vi "[ex ce] Ordinary Differential Equations.vi"(6 "time variable":string="t", 7 "time end":dbl=5.0 format="%.2f", 10 "h (time step)":dbl=0.001 min=0.0 format="%.4f", 11 "time start":dbl format="%.2f") -> (1 "GMath ticks":u32 caption="ms")   [LabVIEW 2021]
doc: "CE-Math example.\n\n::: CalcExpress Toolkit :::\nCopyright (c) 2000-2026 Konstantin Shifershteyn. All rights reserved."
uses:
  ce exmpl - 2D difference info.ctl
  <vilib>/gmath/NI_Gmath.lvlib
panel:
  out "max relative difference":T1 {"relative difference, %" format="%#.6g"; "absolute difference" format="%#.6g"}
  out "max absolute difference":T1 {"relative difference, %" format="%#.6g"; "absolute difference" format="%#.6g"}
  in  "stop":bool
  in  "calc":bool
  in  "example":u16(ring) items=["three equations", "two equations", "one equation"]
  out "speed ratio":dbl format="%.3f"
  out "CE stat":string
  out "GM stat":string
  in  "method":enum16{"Runge Kutta", "Euler"}(ring)
  in  "equation parameters":T2(array[cluster])=[{"variable"="x", "formula"="10*(y-x)", "init value"=1.0}, {"variable"="y", "formula"="x*(28-z)-y", "init value"=1.0}, {"variable"="z", "formula"="x*y-(8/3)*z", "init value"=1.0}] {"init value" format="%.2f"}
  out "CalcExpress ticks":u32 caption="ms"
  out "CE data":cluster{dbl[], dbl[]}[](graph) caption="CalcExpress solution"
  out "GM data":cluster{dbl[], dbl[]}[](graph) caption="G Math solution"
  # "NOTE    CalcExpress uses (^) operator to perform bitwise-XOR operation but not exponentiation operation.\nYou have to use double-asterisk (**) operator to compute an exponent in a CalcExpress expression. For sample, x**y ."
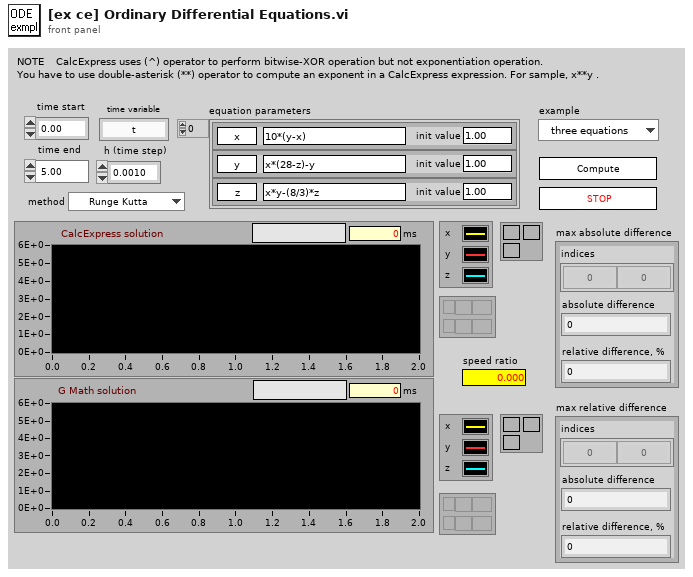
[diagram p1: front panel]
types:
  T1 = typedef "ce exmpl - 2D difference info.ctl" = cluster{"indices":i32[], "absolute difference":dbl, "relative difference, %":dbl}
  T2 = cluster{"variable":string, "formula":string, "init value":dbl}[]
  T3 = cluster{"indexes":i32[], "absolute difference":dbl, "relative difference, %":dbl}
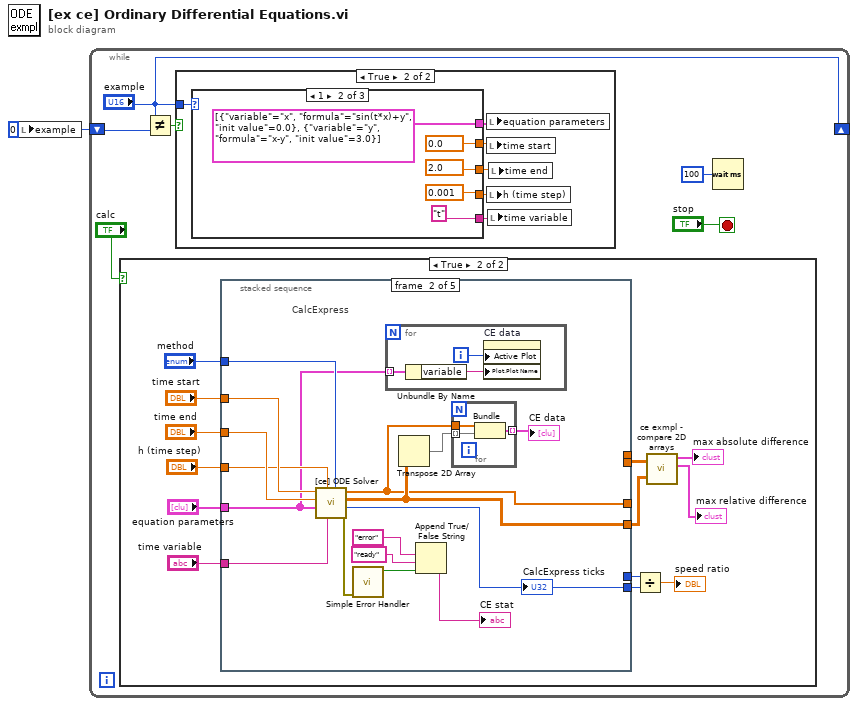
[diagram p0: block diagram]
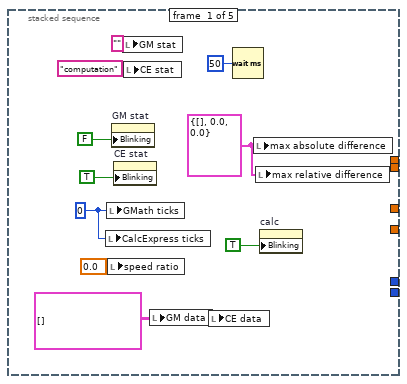
[diagram p3: hidden frame]
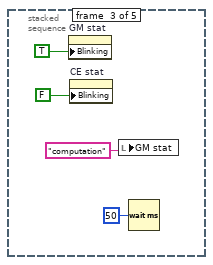
[diagram p4: hidden frame]
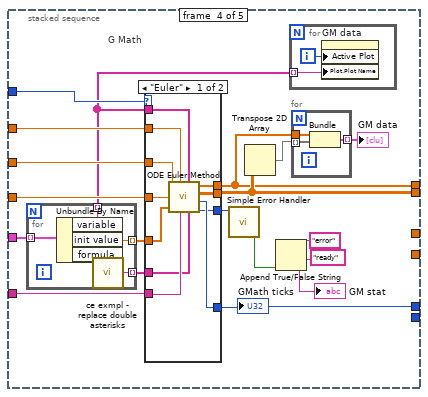
[diagram p5: hidden frame]
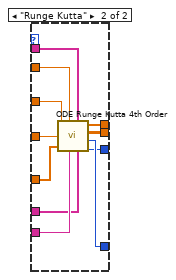
[diagram p6: hidden frame]
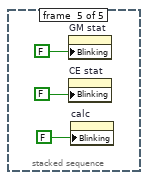
[diagram p7: hidden frame]
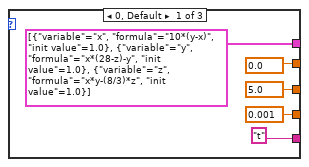
[diagram p9: hidden frame]
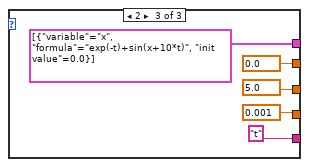
[diagram p10: hidden frame]
diagram:
  w1 = u16 0
  n1 = local write "example"(w1) -> ()
  n2 = while {
    shift-left: w1 -> [w7]
    shift-right: ["example"] -> _
    stop <- "stop" stop-if-true
    n3 = case shown="True" "calc" {
      frame False {
      }
      frame True {
        n4 = stacked-sequence {
          tunnel: "h (time step)" -> [_ w36 _ w75 _]
          tunnel: "time variable" -> [_ w44 _ w74 _]
          tunnel: [_ _ _ w59 _] -> _
          tunnel: "method" -> [_ w46 _ w73 _]
          tunnel: [_ _ _ w60 _] -> w16
          tunnel: "time start" -> [_ w38 _ w72 _]
          tunnel: "time end" -> [_ w37 _ w71 _]
          tunnel: [_ w33 _ _ _] -> _
          tunnel: [_ w34 _ _ _] -> w8
          tunnel: "equation parameters" -> [_ w31 _ w70 _]
          tunnel: [_ _ _ w64 _] -> w13
          tunnel: [_ w39 _ _ _] -> w12
          frame #0 {
            w22 = T3 {"indexes"=[], "absolute difference"=0.0, "relative difference, %"=0.0} ("max absolute difference")
            w23 = cluster{dbl[], dbl[]}[] [] ("GM data")
            w28 = u32 0 ("GMath ticks")
            n5 = local write "CalcExpress ticks"(w28) -> ()
            n6 = local write "GMath ticks"(w28) -> ()
            n7 = local write "speed ratio"(0.0 ("speed ratio")) -> ()
            n8 = property on="GM stat" class="Str"("Blinking"=FALSE ("Write Attribute")) -> ()  [unwired: 2 in, 2 out]
            n9 = property on="CE stat" class="Str"("Blinking"=TRUE ("Write Attribute")) -> ()  [unwired: 2 in, 2 out]
            n10 = local write "GM stat"("" ("CE stat")) -> ()
            n11 = local write "CE stat"("computation" ("GM stat")) -> ()
            n12 = local write "GM data"(w23) -> ()
            n13 = local write "CE data"(w23) -> ()
            n14 = Wait (ms)(milliseconds to wait=u32 50) -> ()  [unwired: 1 out]
            n15 = local write "max absolute difference"(w22) -> ()
            n16 = local write "max relative difference"(w22) -> ()
            n17 = property on="calc" class="Bool"("Blinking"=TRUE ("Write Attribute")) -> ()  [unwired: 2 in, 2 out]
          }
          frame #1 {
            # "CalcExpress"
            n18 = call "[ce] ODE Solver.vi"("method (R-K)"=w46, "time"=w44, "h (step rate)"=w36, "equation descriptions"=w31, "time end"=w37, "time start"=w38) -> ("error out"=w45:errorcluster, "ticks"=w39:u32, "X Values (solution)"=w34:dbl[][], "Times"=w33:dbl[])  [unwired: 2 in]
            "CalcExpress ticks" <- w39
            n19 = call <vilib>:"Simple Error Handler.vi"("error in (no error)"=w45) -> ("error?"=w43:bool)  [unwired: 4 in, 4 out]
            n20 = for {
              tunnel: w31 -> [w47] mode=indexing
              i -> [w49]
              n21 = Unbundle By Name(w47) -> ("variable"=w48:string)
              n22 = property on="CE data" class="XYGraph (strict)"("Active Plot"=w49, "Plot.Plot Name"=w48) -> ()  [unwired: 2 in, 2 out]
            }
            n23 = Transpose 2D Array(2D array=w34) -> (transposed array=w35:dbl[][])
            n24 = Append True/False String(1:w43, 2:"ready" ("false string"), 3:"error" ("true string")) -> (0:→"CE stat":string)  [unwired: 1 in]
            n25 = for {
              tunnel: w33 -> [w52]
              tunnel: w35 -> [w51] mode=indexing
              tunnel: [w50] -> w32 mode=indexing
              n26 = Bundle("Times"=w52, w51) -> (w50:cluster{"Times":dbl[], dbl[]})  [unwired: 1 in]
            }
            "CE data" <- w32
          }
          frame #2 {
            n27 = property on="GM stat" class="Str"("Blinking"=TRUE ("Write Attribute")) -> ()  [unwired: 2 in, 2 out]
            n28 = property on="CE stat" class="Str"("Blinking"=FALSE ("Write Attribute")) -> ()  [unwired: 2 in, 2 out]
            n29 = local write "GM stat"("computation" ("CE stat")) -> ()
            n30 = Wait (ms)(milliseconds to wait=u32 50) -> ()  [unwired: 1 out]
          }
          frame #3 {
            # "G Math"
            n31 = for {
              tunnel: w70 -> [w85] mode=indexing
              tunnel: [w84] -> w69 mode=indexing
              tunnel: [w83] -> w58 mode=indexing
              tunnel: [w82] -> w57 mode=indexing
              n32 = Unbundle By Name(w85) -> ("variable"=w83:string, "init value"=w84:dbl, "formula"=w81:string)
              n33 = call "ce exmpl - replace double asterisks .vi"("formula in"=w81) -> ("formula out"=w82:string)  [unwired: 4 in]
            }
            n34 = case shown="\"Euler\"" w73 {
              tunnel: w72 -> [w96 w107]
              tunnel: w71 -> [w95 w106]
              tunnel: w75 -> [w94 w105]
              tunnel: w74 -> [w93 w104]
              tunnel: [w90 w101] -> w64
              tunnel: [w92 w103] -> w59
              tunnel: [w91 w102] -> w60
              tunnel: w69 -> [w89 w99]
              tunnel: w57 -> [w88 w98]
              tunnel: w58 -> [w87 w100]
              tunnel: [w86 w97] -> w66
              frame "Euler" {
                n35 = call <vilib>:"ODE Euler Method.vi"("time end"=w95, "time start"=w96, "h (step rate)"=w94, "X0"=w89, "time"=w93, "X (name of variables)"=w87, "F(X,t) (right sides of the ODE\nas functions of X and t)"=w88) -> ("Times"=w92:dbl[], "X Values (solution)"=w91:dbl[][], "ticks"=w90:u32, "error"=w86:i32)
              }
              frame "Runge Kutta" {
                n36 = call <vilib>:"ODE Runge Kutta 4th Order.vi"("time end"=w106, "time start"=w107, "h (step rate)"=w105, "X0"=w99, "time"=w104, "X (name of variables)"=w100, "F(X,t) (right sides of the ODE\nas functions of X and t)"=w98) -> ("Times"=w103:dbl[], "X Values (solution)"=w102:dbl[][], "ticks"=w101:u32, "error"=w97:i32)
              }
            }
            "GMath ticks" <- w64
            n37 = call <vilib>:"Simple Error Handler.vi"("error code (no error:0)"=w66) -> ("error?"=w65:bool)  [unwired: 4 in, 4 out]
            n38 = Transpose 2D Array(2D array=w60) -> (transposed array=w61:dbl[][])
            n39 = Append True/False String(1:w65, 2:"ready" ("false string"), 3:"error" ("true string")) -> (0:→"GM stat":string)  [unwired: 1 in]
            n40 = for {
              tunnel: w58 -> [w76] mode=indexing
              i -> [w77]
              n41 = property on="GM data" class="XYGraph (strict)"("Active Plot"=w77, "Plot.Plot Name"=w76) -> ()  [unwired: 2 in, 2 out]
            }
            n42 = for {
              tunnel: w59 -> [w80]
              tunnel: w61 -> [w79] mode=indexing
              tunnel: [w78] -> w62 mode=indexing
              n43 = Bundle("Times"=w80, w79) -> (w78:cluster{"Times":dbl[], dbl[]})  [unwired: 1 in]
            }
            "GM data" <- w62
          }
          frame #4 {
            n44 = property on="GM stat" class="Str"("Blinking"=FALSE ("Write Attribute")) -> ()  [unwired: 2 in, 2 out]
            n45 = property on="CE stat" class="Str"("Blinking"=FALSE ("Write Attribute")) -> ()  [unwired: 2 in, 2 out]
            n46 = property on="calc" class="Bool"("Blinking"=FALSE ("Write Attribute")) -> ()  [unwired: 2 in, 2 out]
          }
        }
        n47 = Divide(x=w13, y=w12) -> (x/y=→"speed ratio":dbl)
        n48 = call "ce exmpl - compare 2D arrays.vi"("array for checking"=w8, "standard array"=w16) -> ("max relative difference"=→"max relative difference":T1, "max absolute difference"=→"max absolute difference":T1)  [unwired: 1 in, 2 out]
      }
    }
    n49 = Not Equal?(x="example", y=w7) -> (x != y?=w3:bool)
    n50 = case shown="True" w3 {
      tunnel: "example" -> [_ w116]
      frame False {
      }
      frame True {
        n51 = case shown="1" w116 {
          tunnel: [T2 [{"variable"="x", "formula"="10*(y-x)", "init value"=1.0}, {"variable"="y", "formula"="x*(28-z)-y", "init value"=1.0}, {"variable"="z", "formula"="x*y-(8/3)*z", "init value"=1.0}] ("equation parameters") T2 [{"variable"="x", "formula"="sin(t*x)+y", "init value"=0.0}, {"variable"="y", "formula"="x-y", "init value"=3.0}] ("equation parameters") T2 [{"variable"="x", "formula"="exp(-t)+sin(x+10*t)", "init value"=0.0}] ("equation parameters")] -> w115
          tunnel: [0.0 0.0 0.0] -> w114
          tunnel: [5.0 2.0 5.0] -> w113
          tunnel: [0.001 0.001 0.001] -> w112
          tunnel: ["t" "t" "t"] -> w111
          frame 0, Default {
          }
          frame 1 {
          }
          frame 2 {
          }
        }
        n52 = local write "equation parameters"(w115) -> ()
        n53 = local write "time start"(w114) -> ()
        n54 = local write "h (time step)"(w112) -> ()
        n55 = local write "time variable"(w111) -> ()
        n56 = local write "time end"(w113) -> ()
      }
    }
    n57 = Wait (ms)(milliseconds to wait=u32 100) -> ()  [unwired: 1 out]
  }
